vi "Clone Template.vi"(6 "Selector":i32, 10 "Subsystem Name":string, 11 "Wizard":T1) -> (0 "Success":bool, 1 "Paths":path[](array[path]), 2 "VI Refs":refnum<vi>[](array[refnum]), 3 "Project Refnum":refnum<vi>, 5 "Subsystem Path":path, 7 "Application":refnum<vi>)   [LabVIEW 2023]
uses:
  <resource>/Framework/Providers/API/ItemRef.ctl
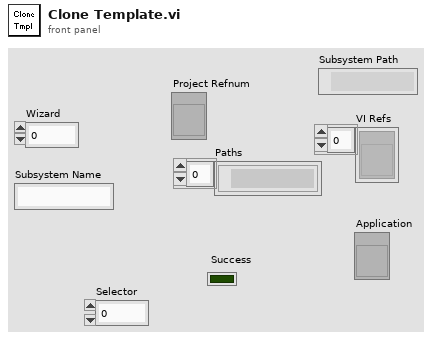
[diagram p1: front panel]
types:
  T1 = typedef "ItemRef.ctl" = u64
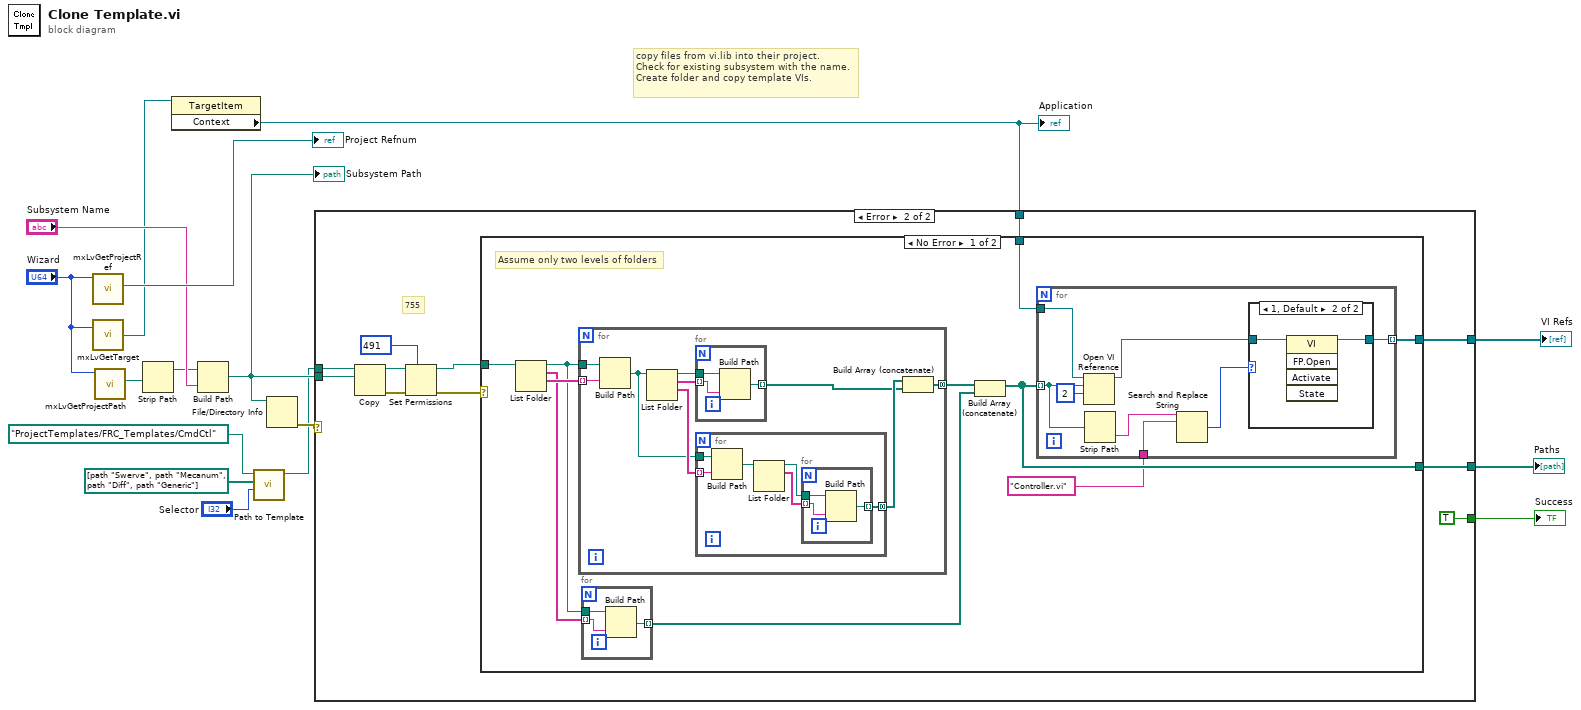
[diagram p0: block diagram]
diagram:
  # "copy files from vi.lib into their project.\nCheck for existing subsystem with the name.\nCreate folder and copy template VIs."
  n1 = call <resource>:"mxLvGetProjectRef.vi"("Item"="Wizard") -> ("Project Refnum"=→"Project Refnum":refnum<vi>)  [unwired: 8 in, 2 out]
  n2 = call <resource>:"mxLvGetTarget.vi"("Item"="Wizard") -> ("Target"=w6:refnum<vi>)  [unwired: 1 in, 2 out]
  n3 = call <resource>:"mxLvGetProjectPath.vi"("Item"="Wizard") -> ("Project Path"=w14:path)  [unwired: 8 in, 2 out]
  n4 = Strip Path(path=w14) -> (stripped path=w13:path)  [unwired: 1 out]
  n5 = property class="TargetItem"(reference=w6) -> ("Context"=w5:refnum<vi>)  [unwired: 1 in, 2 out]
  "Application" <- w5
  n6 = Build Path(base path=w13, name or relative path="Subsystem Name") -> (appended path=w10:path)
  "Subsystem Path" <- w10
  n7 = call <resource>:"Path to Template.vi"("Selector"="Selector", "Array"=path[] [path "Swerve", path "Mecanum", path "Diff", path "Generic"], "Path"=path "ProjectTemplates/FRC_Templates/CmdCtl") -> ("resolved path"=w1:path)  [unwired: 8 in]
  n8 = File/Directory Info(path=w10) -> (error out=w9:errorcluster)  [unwired: 1 in, 6 out]
  n9 = case shown="Error" w9 {
    tunnel: [_ w27] -> w12
    tunnel: w1 -> [_ w26]
    tunnel: [_ w25] -> w11
    tunnel: w10 -> [_ w24]
    tunnel: [_ TRUE] -> w8
    tunnel: w5 -> [_ w22]
    frame No Error {
    }
    frame Error {
      # "755"
      n10 = Copy(10:w24, 11:w26) -> (0:w19:errorcluster, 3:w21:path)  [unwired: 3 in, 1 out]
      n11 = Set Permissions(7:i16 491 ("permissions"), 8:w19, 11:w21) -> (0:w18:errorcluster, 3:w20:path)  [unwired: 2 in]
      n12 = case shown="No Error" w18 {
        tunnel: w20 -> [w37 _]
        tunnel: [w31 _] -> w27
        tunnel: [w30 _] -> w25
        tunnel: w22 -> [w29 _]
        frame No Error {
          # "Assume only two levels of folders"
          n13 = List Folder(path=w37) -> (path out=w35:path, filenames=w34:string[], folder names=w36:string[])  [unwired: 3 in, 1 out]
          n14 = for {
            tunnel: w36 -> [w59] mode=indexing
            tunnel: w35 -> [w60]
            tunnel: [w54] -> w33 mode=concatenating
            n15 = Build Path(base path=w60, name or relative path=w59) -> (appended path=w55:path)
            n16 = List Folder(path=w55) -> (path out=w58:path, filenames=w57:string[], folder names=w56:string[])  [unwired: 3 in, 1 out]
            n17 = for {
              tunnel: w58 -> [w72]
              tunnel: w57 -> [w71] mode=indexing
              tunnel: [w70] -> w52 mode=indexing
              n18 = Build Path(base path=w72, name or relative path=w71) -> (appended path=w70:path)
            }
            n19 = for {
              tunnel: w56 -> [w65] mode=indexing
              tunnel: w55 -> [w64]
              tunnel: [w61] -> w53 mode=concatenating
              n20 = Build Path(base path=w64, name or relative path=w65) -> (appended path=w66:path)
              n21 = List Folder(path=w66) -> (path out=w63:path, filenames=w62:string[])  [unwired: 3 in, 2 out]
              n22 = for {
                tunnel: w63 -> [w69]
                tunnel: w62 -> [w68] mode=indexing
                tunnel: [w67] -> w61 mode=indexing
                n23 = Build Path(base path=w69, name or relative path=w68) -> (appended path=w67:path)
              }
            }
            n24 = Build Array (concatenate)(w53, w52) -> (w54:path[])
          }
          n25 = for {
            tunnel: w35 -> [w51]
            tunnel: w34 -> [w50] mode=indexing
            tunnel: [w49] -> w32 mode=indexing
            n26 = Build Path(base path=w51, name or relative path=w50) -> (appended path=w49:path)
          }
          n27 = Build Array (concatenate)(w33, w32) -> (w30:path[])
          n28 = for {
            tunnel: w30 -> [w41] mode=indexing
            tunnel: w29 -> [w45]
            tunnel: [w43] -> w31 mode=indexing
            tunnel: "Controller.vi" ("Type") -> [w39]
            n29 = Open VI Reference(application reference (local)=w45, vi path=w41, options=2) -> (vi reference=w44:refnum<vi>)  [unwired: 3 in, 1 out]
            n30 = Strip Path(path=w41) -> (name=w40:string)  [unwired: 1 out]
            n31 = Search and Replace String(input string=w40, search string=w39) -> (number of replacements=w38:i32)  [unwired: 6 in, 3 out]
            n32 = case shown="1, Default" w38 {
              tunnel: w44 -> [w46 w48]
              tunnel: [w46 w47] -> w43
              frame 0 {
              }
              frame 1, Default {
                n33 = invoke class="VI" method="FP.Open"(reference=w48) -> (reference out=w47:refnum<vi>)  [unwired: 4 in, 4 out]
              }
            }
          }
        }
        frame Error {
        }
      }
    }
  }
  "VI Refs" <- w12
  "Paths" <- w11
  "Success" <- w8
